vi "Own20261012_GetFormulaInfo.vi"() -> ()   [LabVIEW 2024]
panel:
  out "error out":errorcluster caption="错误输出"
  out "parameter_ids":refnum<vi>[](array[refnum])
  out "expression":string
  in  "formula_id":u32
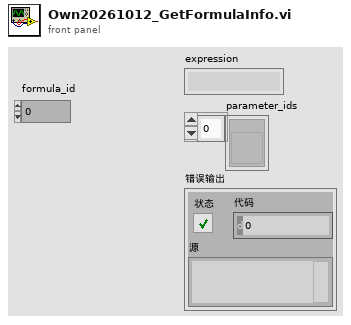
[diagram p1: front panel]
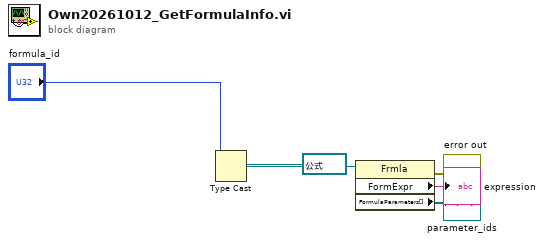
[diagram p0: block diagram]
diagram:
  n1 = Type Cast(type=refnum<vi> refnum ("引用"), x="formula_id") -> (*(type *) &x=w4:refnum<vi>)
  n2 = property class="Frmla"(reference=w4) -> (error out=→"error out":errorcluster, "FormExpr"=→"expression":string, "FormulaParameters[]"=→"parameter_ids":refnum<vi>[])  [unwired: 1 in, 1 out]
